vi "Select Next Path.vi"(0 "Auto Data":T1) -> (1 "Command Info":T3(array[cluster]), 3 "Current Limits":dbl, 4 "Velocities":T2[](array[typedef]), 6 "Positions":cluster{"x":dbl, "y":dbl, "th":dbl}[](array[cluster]), 8 "Number of Remaining Auto Paths":dbl, 10 "Zero Velocity?":bool[](array[boolean]), 13 "Name of Path":string, 14 "Auto Data Out":T1, 15 "Zero Translational Velocity?":bool[](array[boolean]))   [LabVIEW 2023]
uses:
  swerve-template/Type Definitions/Data/Robot Velocities.ctl
  Implementation/Auto Data.ctl
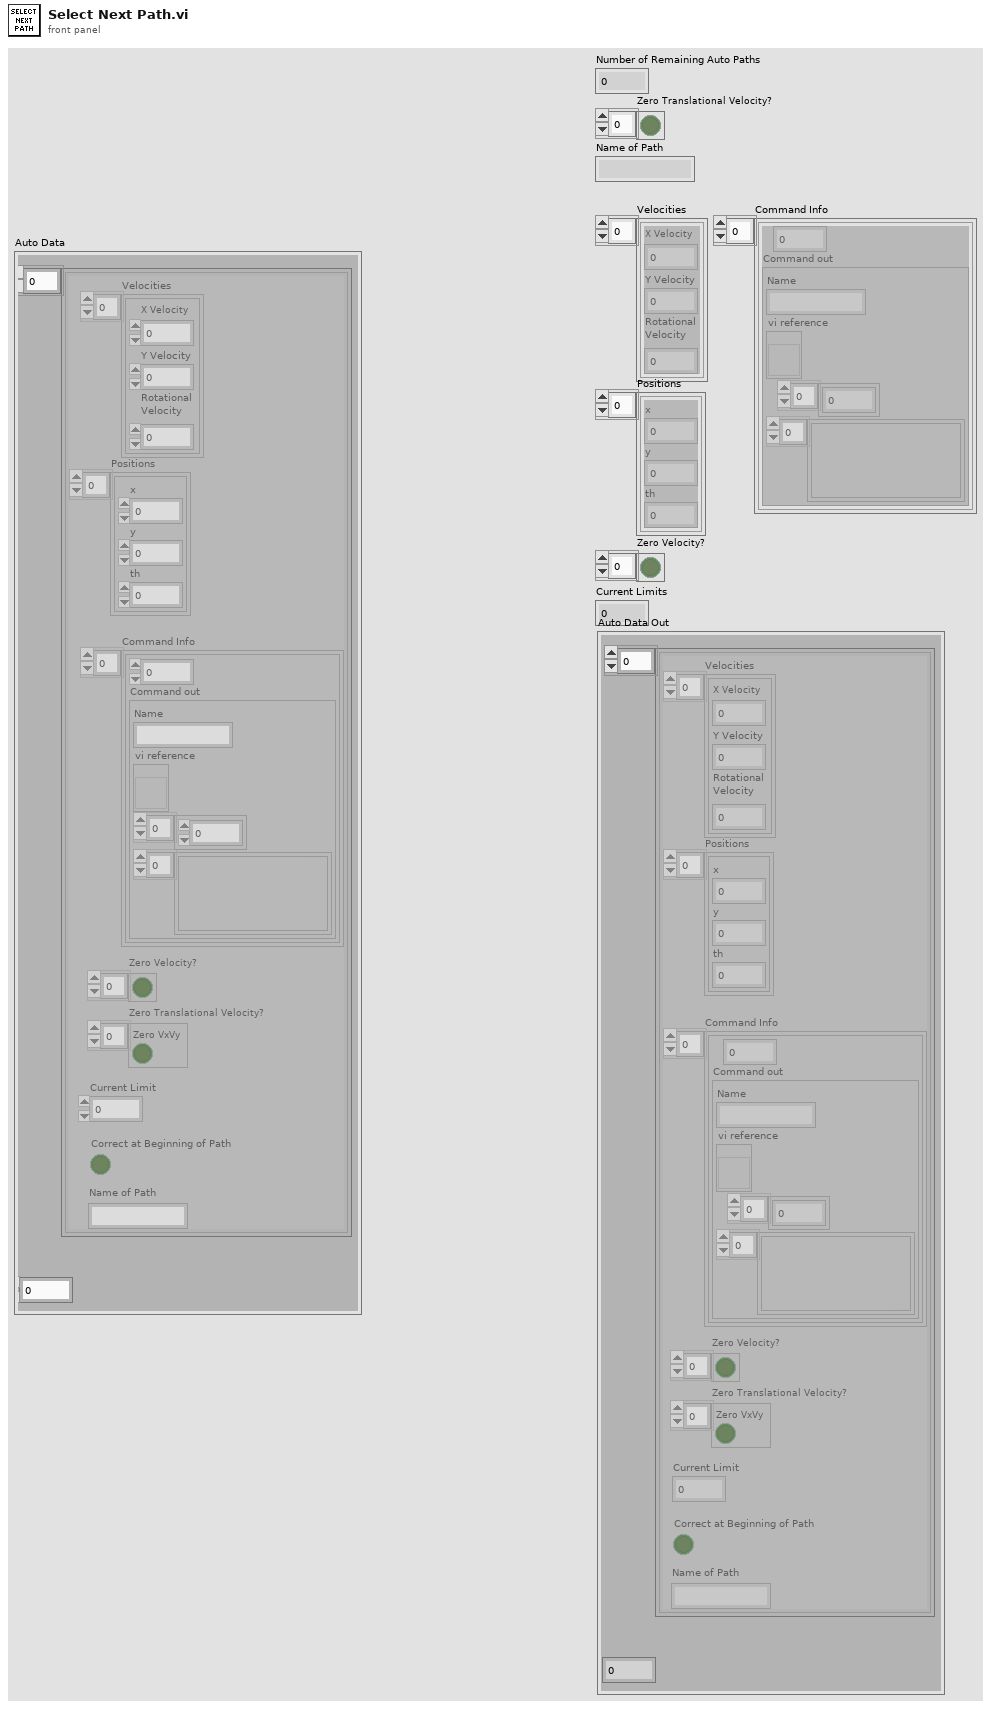
[diagram p1: front panel]
types:
  T1 = typedef "Auto Data.ctl" = cluster{"Auto Data":cluster{"Velocities":T2[], "Positions":cluster{"x":dbl, "y":dbl, "th":dbl}[], "Command Info":cluster{dbl, "Command out":cluster{"Name":string, "vi reference":refnum<vi>, i32[], variant[]}}[], "Zero Velocity?":bool[], "Zero Translational Velocity?":bool[], "Current Limit":dbl, "Correct at Beginning of Path":bool, "Name of Path":string}[], "Number of Remaining Auto Paths":dbl}
  T2 = typedef "Robot Velocities.ctl" = cluster{"X Velocity":dbl, "Y Velocity":dbl, "Rotational \nVelocity":dbl}
  T3 = cluster{dbl, "Command out":cluster{"Name":string, "vi reference":refnum<vi>, i32[], variant[]}}[]
  T4 = cluster{"Velocities":T2[], "Positions":cluster{"x":dbl, "y":dbl, "th":dbl}[], "Command Info":cluster{dbl, "Command out":cluster{"Name":string, "vi reference":refnum<vi>, i32[], variant[]}}[], "Zero Velocity?":bool[], "Zero Translational Velocity?":bool[], "Current Limit":dbl, "Correct at Beginning of Path":bool, "Name of Path":string}[]
  T5 = cluster{"Velocities":T2[], "Positions":cluster{"x":dbl, "y":dbl, "th":dbl}[], "Command Info":cluster{dbl, "Command out":cluster{"Name":string, "vi reference":refnum<vi>, i32[], variant[]}}[], "Zero Velocity?":bool[], "Zero Translational Velocity?":bool[], "Current Limit":dbl, "Correct at Beginning of Path":bool, "Name of Path":string}
  T6 = cluster{cluster{"Velocities":T2[], "Positions":cluster{"x":dbl, "y":dbl, "th":dbl}[], "Command Info":cluster{dbl, "Command out":cluster{"Name":string, "vi reference":refnum<vi>, i32[], variant[]}}[], "Zero Velocity?":bool[], "Zero Translational Velocity?":bool[], "Current Limit":dbl, "Correct at Beginning of Path":bool, "Name of Path":string}[], dbl}
  T7 = cluster{"Auto Data":cluster{"Velocities":T2[], "Positions":cluster{"x":dbl, "y":dbl, "th":dbl}[], "Command Info":cluster{dbl, "Command out":cluster{"Name":string, "vi reference":refnum<vi>, i32[], variant[]}}[], "Zero Velocity?":bool[], "Zero Translational Velocity?":bool[], "Current Limit":dbl, "Correct at Beginning of Path":bool, "Name of Path":string}[], "Number of Remaining Auto Paths":dbl}
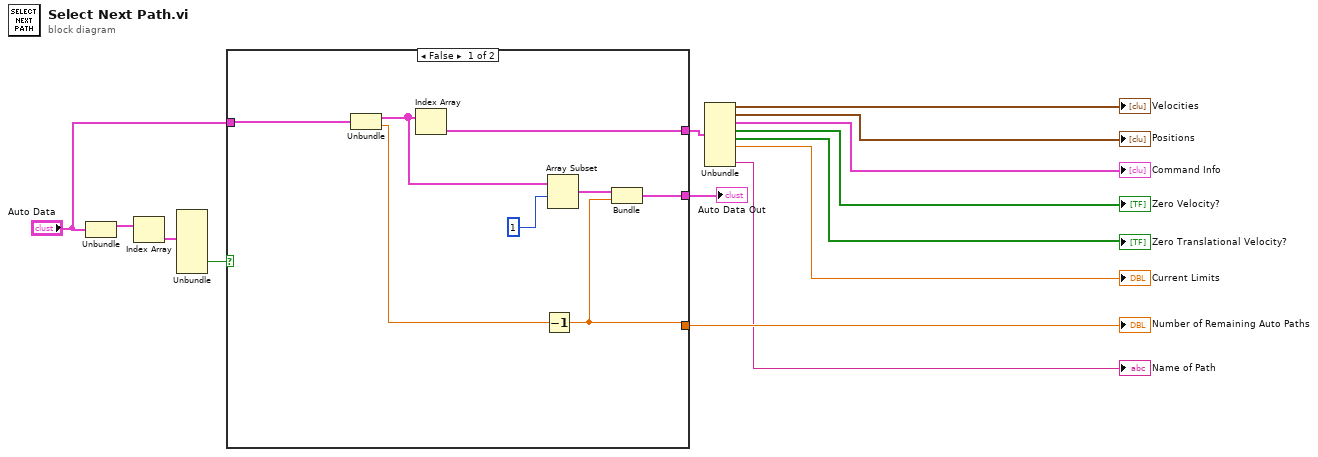
[diagram p0: block diagram]
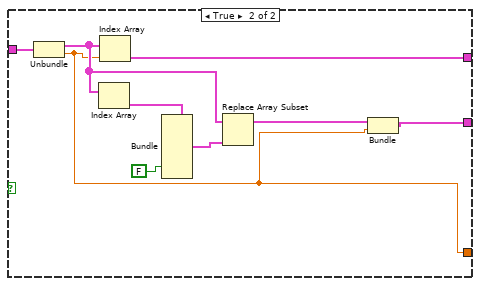
[diagram p2: hidden frame]
diagram:
  n1 = Unbundle("Auto Data") -> ("Auto Data"=w12:T4)  [unwired: 1 out]
  n2 = Index Array(array=w12) -> (element=w11:T5)  [unwired: 1 in]
  n3 = Unbundle(w11) -> ("Correct at Beginning of Path"=w10:bool)  [unwired: 7 out]
  n4 = case shown="False" w10 {
    tunnel: "Auto Data" -> [w22 w31]
    tunnel: [w21 w30] -> w14
    tunnel: [w18 w23] -> w9
    tunnel: [w16 w24] -> w2
    frame False {
      n5 = Unbundle(w22) -> ("Auto Data"=w19:T4, "Number of Remaining Auto Paths"=w20:dbl)
      n6 = Index Array(array=w19) -> (element=w21:T5)  [unwired: 1 in]
      n7 = Decrement(x=w20) -> (x-1=w18:dbl)
      n8 = Array Subset(array=w19, index=1) -> (w17:T4)  [unwired: 1 in]
      n9 = Bundle(w17, w18) -> (w16:T6)  [unwired: 1 in]
    }
    frame True {
      n10 = Unbundle(w31) -> ("Auto Data"=w26:T4, "Number of Remaining Auto Paths"=w23:dbl)
      n11 = Index Array(array=w26) -> (element=w29:T5)  [unwired: 1 in]
      n12 = Index Array(array=w26, index=w23) -> (element=w30:T5)
      n13 = Bundle(cluster=w29, "Correct at Beginning of Path"=FALSE) -> (w27:T5)  [unwired: 7 in]
      n14 = Replace Array Subset(array=w26, new element=w27) -> (w25:T4)  [unwired: 1 in]
      n15 = Bundle("Auto Data"=w25, "Number of Remaining Auto Paths"=w23) -> (w24:T7)  [unwired: 1 in]
    }
  }
  "Number of Remaining Auto Paths" <- w9
  "Auto Data Out" <- w2
  n16 = Unbundle(w14) -> ("Velocities"=→"Velocities":T2[], "Positions"=→"Positions":cluster{"x":dbl, "y":dbl, "th":dbl}[], "Command Info"=→"Command Info":T3, "Zero Velocity?"=→"Zero Velocity?":bool[], "Zero Translational Velocity?"=→"Zero Translational Velocity?":bool[], "Current Limit"=→"Current Limits":dbl, "Name of Path"=→"Name of Path":string)  [unwired: 1 out]
